vi "Global Log To String(Source Time).vi"(6 "Format String":string="%<%H:%M:%S%3u>T", 10 "Log":T1) -> (3 "Log String":string)   [LabVIEW 2017, in "Communicable State Machine.lvlib"]
doc: "Converts global log data clusters to strings, using the send time as the timestamp.\n\n-- <b>Controls</b> --\n- <b>Log</b>: Global log data cluster.\n- <b>Format String</b>: Timestamp format.\n\n-- <b>Indicators</b> --\n- <b>Log String</b>: Global log string."
uses:
  Communicable State Machine.lvlib
  _Support/Typedef/_CSM_GlobalLog_MSG.ctl
  _Support/Typedef/_CSM_Response Source Message.ctl
  _Support/Typedef/_CSM_GlobalLog_MSG_TYPE.ctl
  _Shared/CSM Shared.lvlib
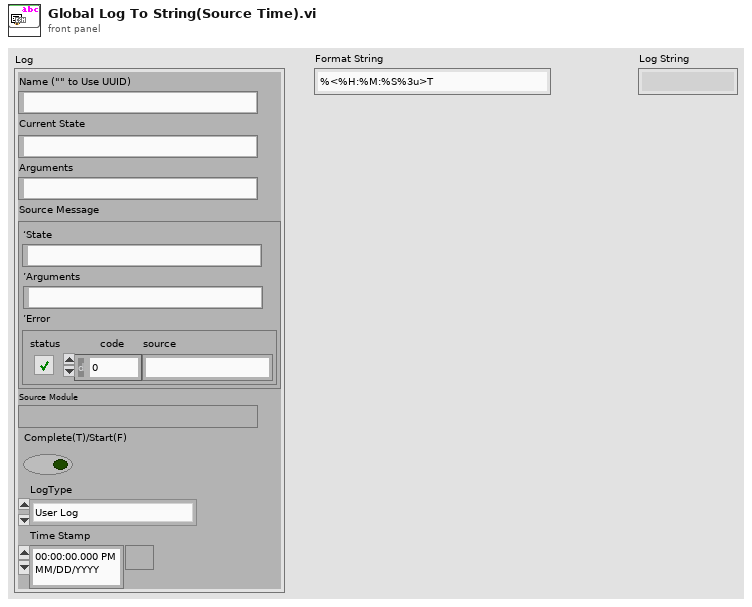
[diagram p1: front panel]
types:
  T1 = typedef "Communicable State Machine.lvlib/_CSM_GlobalLog_MSG.ctl" = cluster{"Name (\"\" to Use UUID)":string, "Current State":string, "Arguments":string, "Source Message":T2, "Source Module":string, "Complete(T)/Start(F)":bool, "LogType":T3, "Time Stamp":timestamp}
  T2 = typedef "Communicable State Machine.lvlib/_CSM_Response Source Message.ctl" = cluster{"‘State":string, "’Arguments":string, "’Error":errorcluster}
  T3 = typedef "Communicable State Machine.lvlib/_CSM_GlobalLog_MSG_TYPE.ctl" = enum16{"User Log", "State Change", "Status", "Interrupt", "Register", "Unregister", "Error Log", "Module Created", "Module Destroyed", "Async Message", "No-Rep Async Message", "Sync Message", "AsyncMsg Complete", "SyncMsg Complete"}
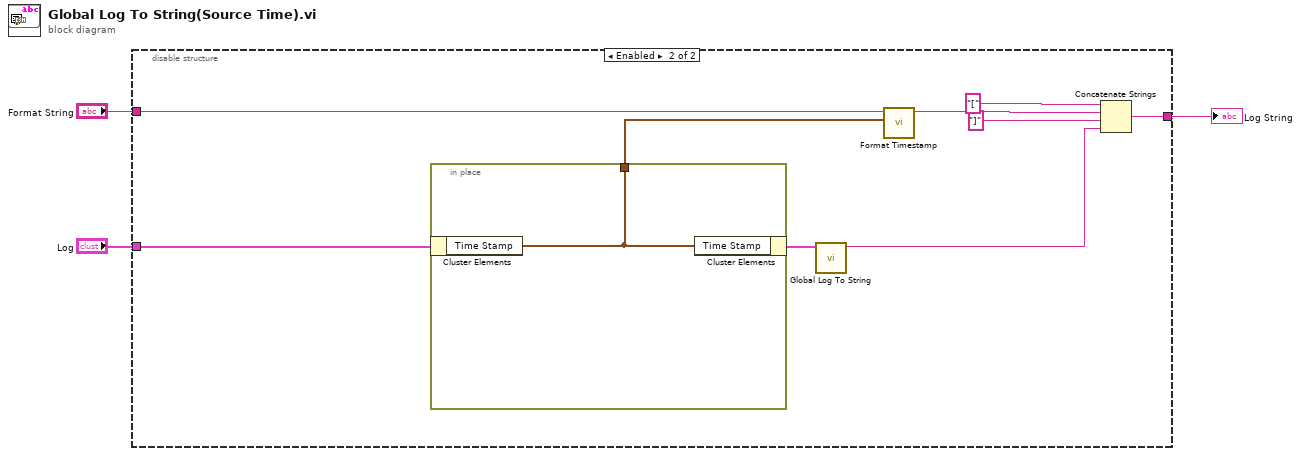
[diagram p0: block diagram]
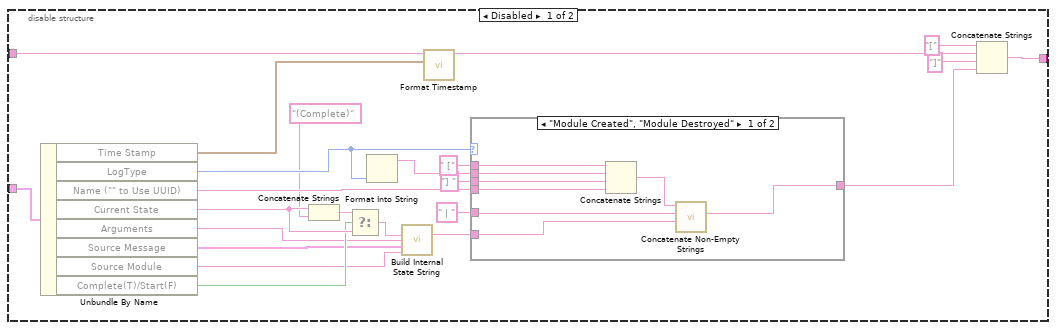
[diagram p2: hidden frame]
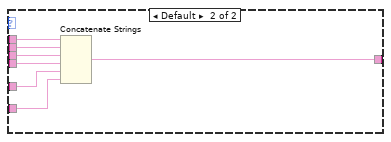
[diagram p3: hidden frame]
diagram:
  n1 = disable-structure "Diagram Disable Structure" shown="Enabled" {
    disable-tunnel: "Log" -> [w15 w45]
    disable-tunnel: "Format String" -> [w10 w50]
    disable-tunnel: [w6 w47] -> w1
    frame Disabled {
      n2 = Unbundle By Name(w15) -> ("Time Stamp"=w11:timestamp, "LogType"=w14:T3, "Name (\"\" to Use UUID)"=w16:string, "Current State"=w23:string, "Arguments"=w17:string, "Source Message"=w18:T2, "Source Module"=w19:string, "Complete(T)/Start(F)"=w21:bool)
      n3 = Concatenate Strings(w23, "(Complete)" ("string")) -> (w22:string)
      n4 = Select(t=w22, s=w21, f=w23) -> (s? t:f=w24:string)
      n5 = Format Into String(w14) -> (resulting string=w13:string)  [unwired: 3 in, 1 out]
      n6 = call "Build Internal State String.vi"("State"=w24, "Arguments (\"\")"=w17, "Additional Information"=w18, "Source (\"\")"=w19) -> ("State With Arguments"=w20:string)  [unwired: 11 in]
      n7 = call "Format Timestamp.vi"("Timestamp"=w11, "Format String"=w10) -> ("String"=w5:string)  [unwired: 9 in]
      n8 = case shown="\"Module Created\", \"Module Destroyed\"" w14 {
        tunnel: w13 -> [w33 w41]
        tunnel: "] " ("string") -> [w32 w40]
        tunnel: " [" ("string") -> [w34 w39]
        tunnel: w16 -> [w31 w38]
        tunnel: [w27 w35] -> w7
        tunnel: w20 -> [w29 w36]
        tunnel: " | " ("string") -> [w28 w37]
        frame "Module Created", "Module Destroyed" {
          n9 = Concatenate Strings(w34, w33, w32, w31) -> (w30:string)
          n10 = call "Concatenate Non-Empty Strings.vi"("String2"=w29, "Seperator(Carriage Return)"=w28, "String1"=w30) -> ("Result String"=w27:string)  [unwired: 5 in]
        }
        frame Default {
          n11 = Concatenate Strings(w39, w41, w40, w38, w37, w36) -> (w35:string)
        }
      }
      n12 = Concatenate Strings("[" ("string"), w5, "]" ("string"), w7) -> (w6:string)
    }
    frame Enabled {
      n13 = in-place {
        in-place-border: [w51] -> w44
        n14 = in-place-cluster #1(w45) -> ("Time Stamp"=w51:timestamp)
        n15 = in-place-cluster #1("Time Stamp"=w51) -> (w43:T1)
      }
      n16 = call "Global Log To String.vi"("Log"=w43) -> ("Log String"=w42:string)  [unwired: 9 in]
      n17 = call "Format Timestamp.vi"("Timestamp"=w44, "Format String"=w50) -> ("String"=w46:string)  [unwired: 9 in]
      n18 = Concatenate Strings("[" ("string"), w46, "]" ("string"), w42) -> (w47:string)
    }
  }
  "Log String" <- w1
